vi "XMLCloseConfiguration.vi"(8 "error in (no error)":errorcluster, 10 "OPC UA server refnum in":refnum<k21>, 11 "DOM document in":refnum<k20>) -> (0 "error out":errorcluster, 2 "OPC UA server refnum out":refnum<k21>)   [LabVIEW 2014, in "OPCUA XML(dev).lvlib"]
uses:
  OPCUA XML(dev).lvlib
  <vilib>/xml/NI_XML.lvlib
  <vilib>/xml/Close Reference(Node).vi
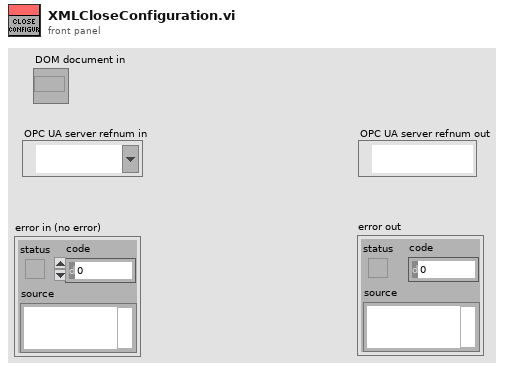
[diagram p1: front panel]
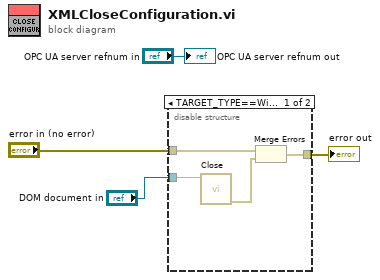
[diagram p0: block diagram]
diagram:
  n1 = disable-structure shown="TARGET_TYPE==Windows" {
    disable-tunnel: "DOM document in" -> [w8 _]
    disable-tunnel: [w6 w9] -> w2
    disable-tunnel: "error in (no error)" -> [w5 w9]
    frame condition #0 {
      n2 = call-poly <vilib>:"Close.vi"("node"=w8) -> ("error out"=w7:errorcluster)  [unwired: 1 in, 7 out]
      n3 = Merge Errors(w5, w7) -> (w6:errorcluster)
    }
    frame condition #1 (active) {
    }
  }
  "error out" <- w2
  "OPC UA server refnum out" <- "OPC UA server refnum in"
